vi "TDMS_ReadFile.vi"(8 "error in (no error)":errorcluster, 11 "file path":path) -> (0 "error out":errorcluster, 3 "data":i16[][](array[numeric]))   [LabVIEW 2025]
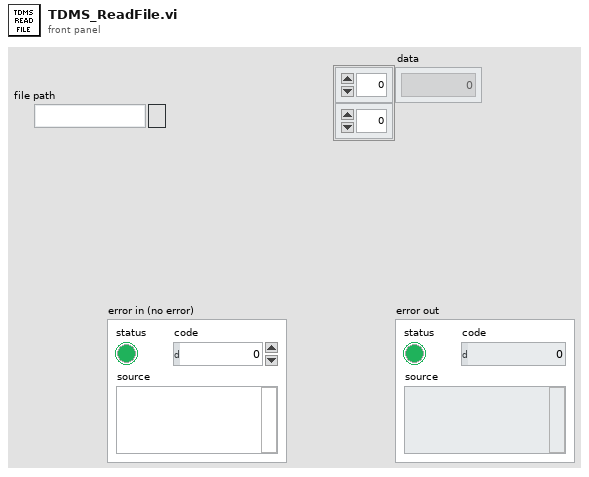
[diagram p1: front panel]
types:
  T1 = enum16{"open", "open or create", "create or replace", "create", "open (read-only)"}
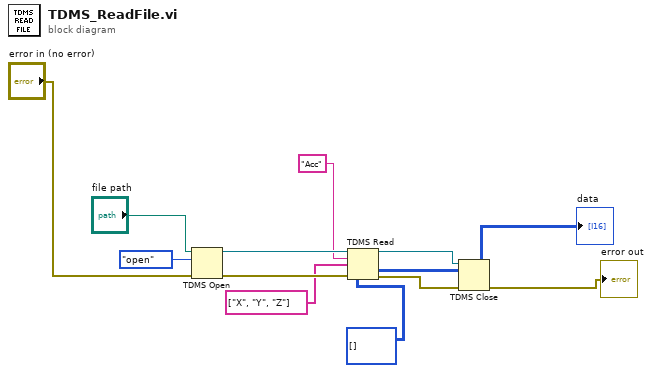
[diagram p0: block diagram]
diagram:
  n1 = TDMS Open(8:"error in (no error)", 10:T1."open" ("operation (0:open)"), 11:"file path") -> (0:w10:errorcluster, 3:w11:refnum<k34>)  [unwired: 4 in]
  n2 = TDMS Read(0:w11, 5:"Acc" ("group name in"), 7:string[] ["X", "Y", "Z"] ("channel name(s) in"), 11:w10, 12:i16[][] []) -> (4:w7:refnum<k34>, 10:→"data":i16[][], 15:w8:errorcluster)  [unwired: 3 in, 3 out]
  n3 = TDMS Close(8:w8, 11:w7) -> (0:→"error out":errorcluster)  [unwired: 1 out]
